vi "Mean Of Pair.vi"(0 "x":i32, 1 "y":i32) -> (2 "Mean":dbl)   [LabVIEW 2026]
doc: "Round20 multi-VI demo subVI (P6): plain arithmetic - Divide x by y. Panel: x in (conIdx0, required), y in (conIdx1, required), Mean out (conIdx2, recommended). Type note measured in this round: int32/int32 through Divide yields DBL, so Mean is double - the caller wires that DBL across its own connector pane, making the int-to-DBL promotion part of the test."
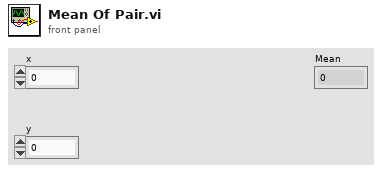
[diagram p1: front panel]
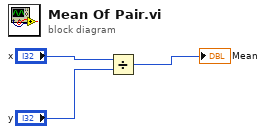
[diagram p0: block diagram]
diagram:
  n1 = Divide(x="x", y="y") -> (x/y=→"Mean":i32)
